vi "test Acyclic Loopback with SDI.vi"(8 "error in":errorcluster, 11 "TestCase in":refnum<class "Single Board Loopback.lvclass">) -> (0 "error out":errorcluster, 3 "TestCase out":refnum<class "Single Board Loopback.lvclass">)   [LabVIEW 2020, in "Single Board Loopback.lvclass"]
uses:
  Single Board Loopback.lvclass
  <vilib>/addons/_JKI Toolkits/VI Tester/TestCase.llb/TestCase.lvclass
  <vilib>/NI VeriStand/Execution/Workspace/NI_VS Workspace ExecutionAPI.lvlib
  <vilib>/NI/VeriStand Custom Device Testing Tools/VeriStandTestUtilities/VeriStandTestUtilities.lvlib
  <vilib>/NI VeriStand/Execution/Workspace/NI VeriStand - Set Single Channel Value.vi
  <vilib>/numeric/Random Number (Range) U64.vi
  C:/Users/nitest/Desktop/Git 2020/niveristand-custom-device-testing-tools/VeriStandTestCase/VeriStandTestCase.lvclass
  C:/Program Files (x86)/National Instruments/LabVIEW 2020/vi.lib/addons/_JKI Toolkits/VI Tester/TestCase.llb/TestCase.lvclass
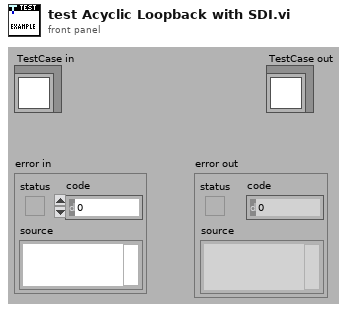
[diagram p1: front panel]
types:
  T1 = typedef "NI_VS Workspace ExecutionAPI.lvlib/WorkspaceAPI.ctl" = refnum<k24>
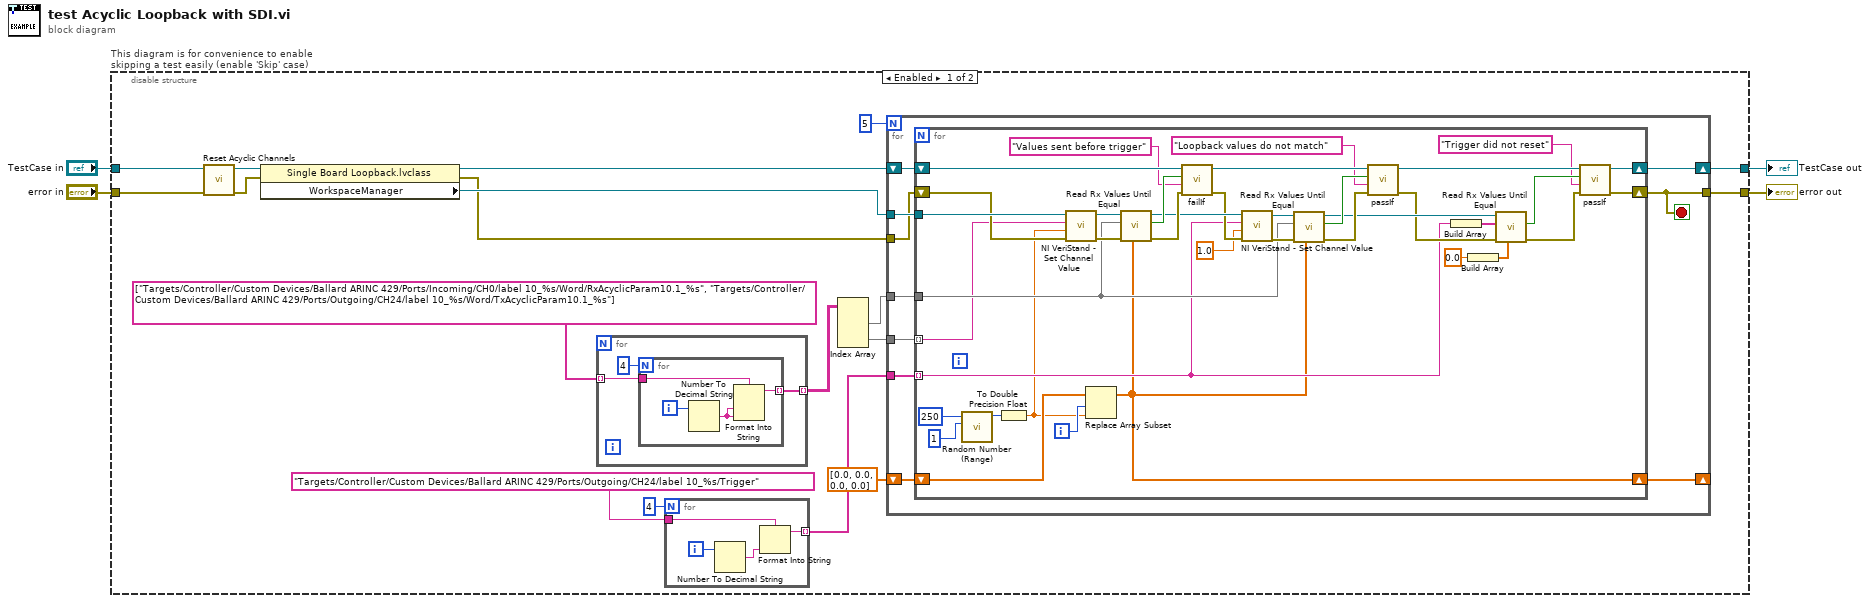
[diagram p0: block diagram]
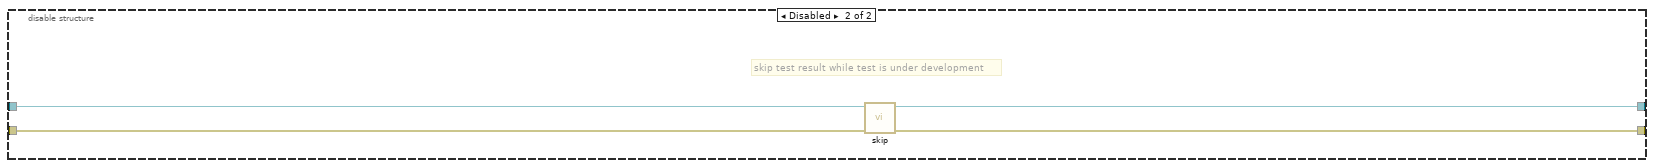
[diagram p2: hidden frame]
diagram:
  n1 = disable-structure "This diagram is for convenience to enable skipping a test easily (enable 'Skip' case)" shown="Enabled" {
    disable-tunnel: "TestCase in" -> [w14 w85]
    disable-tunnel: [w17 w83] -> w1
    disable-tunnel: [w16 w84] -> w3
    disable-tunnel: "error in" -> [w18 w82]
    frame Enabled {
      n2 = call "Reset Acyclic Channels.vi"("error in (no error)"=w18, "reference in"=w14) -> ("error out"=w15:errorcluster, "reference out"=w13:refnum<class "Single Board Loopback.lvclass">)  [unwired: 8 in]
      n3 = property class="Single Board Loopback.lvclass"(reference=w13, error in=w15) -> (reference out=w20:refnum<class "Single Board Loopback.lvclass">, error out=w21:errorcluster, "WorkspaceManager"=w22:T1)
      n4 = for {
        tunnel: [w29] -> w9 mode=indexing
        tunnel: string[] ["Targets/Controller/Custom Devices/Ballard ARINC 429/Ports/Incoming/CH0/label 10_%s/Word/RxAcyclicParam10.1_%s", "Targets/Controller/Custom Devices/Ballard ARINC 429/Ports/Outgoing/CH24/label 10_%s/Word/TxAcyclicParam10.1_%s"] -> [w28] mode=indexing
        n5 = for {
          N: 4 -> [_]
          tunnel: w28 -> [w30]
          tunnel: [w32] -> w29 mode=indexing
          i -> [w33]
          n6 = Number To Decimal String(number=w33) -> (decimal integer string=w31:string)  [unwired: 1 in]
          n7 = Format Into String(format string=w30, w31, w31) -> (resulting string=w32:string)  [unwired: 2 in, 1 out]
        }
      }
      n8 = for {
        N: 4 -> [_]
        tunnel: [w25] -> w6 mode=indexing
        tunnel: "Targets/Controller/Custom Devices/Ballard ARINC 429/Ports/Outgoing/CH24/label 10_%s/Trigger" -> [w23]
        i -> [w26]
        n9 = Number To Decimal String(number=w26) -> (decimal integer string=w24:string)  [unwired: 1 in]
        n10 = Format Into String(format string=w23, w24) -> (resulting string=w25:string)  [unwired: 2 in, 1 out]
      }
      n11 = Index Array(array=w9) -> (element #1=w11:string[], element #2=w10:string[])  [unwired: 4 in]
      n12 = for {
        N: 5 -> [_]
        tunnel: w22 -> [w43]
        tunnel: w21 -> [w41]
        shift-right: [w39] -> w17
        shift-left: w20 -> [w42]
        tunnel: [w40] -> w16
        tunnel: w10 -> [w38]
        tunnel: w6 -> [w37]
        tunnel: w11 -> [w36]
        shift-right: [w35] -> _
        shift-left: dbl[] [0.0, 0.0, 0.0, 0.0] -> [w34]
        stop <- w40 stop-if-true
        n13 = for {
          tunnel: w43 -> [w80]
          shift-right: [w64] -> w39
          shift-left: w42 -> [w76]
          shift-right: [w66] -> w40
          shift-left: w41 -> [w74]
          tunnel: w38 -> [w52] mode=indexing
          tunnel: w37 -> [w51] mode=indexing
          tunnel: w36 -> [w53]
          shift-right: [w46] -> w35
          shift-left: w34 -> [w47]
          i -> [w45]
          n14 = call-poly <vilib>:"Random Number (Range).vi"("lower bound (0)"=u64 1 ("upper bound (100)"), "upper bound (100)"=u64 250) -> ("number"=w56:u64)  [unwired: 9 in]
          n15 = To Double Precision Float(number=w56) -> (double precision float=w44:dbl)
          n16 = call-poly <vilib>:"NI VeriStand - Set Channel Value.vi"("error in (no error)"=w74, "Value"=w44, "Channel"=w52, "WorkspaceManager in"=w80) -> ("error out"=w77:errorcluster, "WorkspaceManager out"=w79:T1)  [unwired: 6 in]
          n17 = Replace Array Subset(array=w47, new element=w44, index=w45) -> (w46:dbl[])
          n18 = call <vilib>:"Read Rx Values Until Equal.vi"("expected values"=w46, "error in"=w77, "Rx aliases"=w53, "workspace manager in"=w79) -> ("error out"=w78:errorcluster, "values equal expected"=w75:bool, "workspace manager out"=w73:T1)  [unwired: 5 in]
          n19 = call-dynamic "failIf.vi"("error in (no error)"=w78, "message (\"\")"="Values sent before trigger" ("message (\"\")"), "fail"=w75, "TestCase in"=w76) -> ("error out"=w72:errorcluster, "TestCase out"=w67:refnum<class "Single Board Loopback.lvclass">)  [unwired: 6 in]
          n20 = call-poly <vilib>:"NI VeriStand - Set Channel Value.vi"("error in (no error)"=w72, "Value"=1.0, "Channel"=w51, "WorkspaceManager in"=w73) -> ("error out"=w70:errorcluster, "WorkspaceManager out"=w71:T1)  [unwired: 6 in]
          n21 = call <vilib>:"Read Rx Values Until Equal.vi"("expected values"=w46, "error in"=w70, "Rx aliases"=w53, "workspace manager in"=w71) -> ("error out"=w68:errorcluster, "values equal expected"=w69:bool, "workspace manager out"=w62:T1)  [unwired: 5 in]
          n22 = call-dynamic "passIf.vi"("error in (no error)"=w68, "message (\"\")"="Loopback values do not match" ("message (\"\")"), "pass"=w69, "TestCase in"=w67) -> ("error out"=w61:errorcluster, "TestCase out"=w65:refnum<class "Single Board Loopback.lvclass">)  [unwired: 6 in]
          n23 = Build Array(w51) -> (w50:string[])
          n24 = Build Array(0.0) -> (w48:dbl[])
          n25 = call <vilib>:"Read Rx Values Until Equal.vi"("expected values"=w48, "error in"=w61, "Rx aliases"=w50, "workspace manager in"=w62) -> ("error out"=w60:errorcluster, "values equal expected"=w63:bool)  [unwired: 5 in, 1 out]
          n26 = call-dynamic "passIf.vi"("error in (no error)"=w60, "message (\"\")"="Trigger did not reset" ("message (\"\")"), "pass"=w63, "TestCase in"=w65) -> ("error out"=w66:errorcluster, "TestCase out"=w64:refnum<class "Single Board Loopback.lvclass">)  [unwired: 6 in]
        }
      }
    }
    frame Disabled {
      # "skip test result while test is under development"
      n27 = call <vilib>:"skip.vi"("error in (no error)"=w82, "TestCase in"=w85) -> ("error out"=w84:errorcluster, "TestCase out"=w83:refnum<class "Single Board Loopback.lvclass">)  [unwired: 8 in]
    }
  }
  "error out" <- w3
  "TestCase out" <- w1
